vi "VIH Platform - Windows - SHELL Error Handler.vi"(8 "error in":errorcluster, 11 "SHELL Error Code":i32) -> (0 "error out":errorcluster)   [LabVIEW 2014]
doc: "::: VI Helpeks :::\nCopyright (c) 2000-2026 Konstantin Shifershteyn. All rights reserved."
panel:
  # "VI Helpeks\nCopyright (c) 2012-2026 Konstantin Shifershteyn"
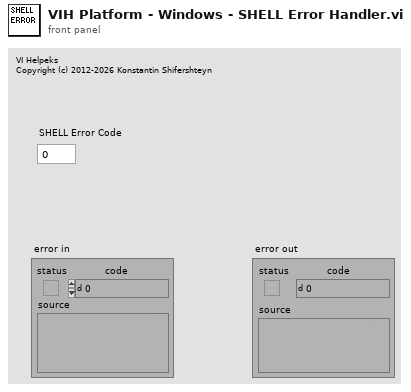
[diagram p1: front panel]
types:
  T1 = cluster{"Product Name":string, "Short Name":string, "Product Version":string, "Release Timestamp":string, "Developer":string, "Copyright":string}
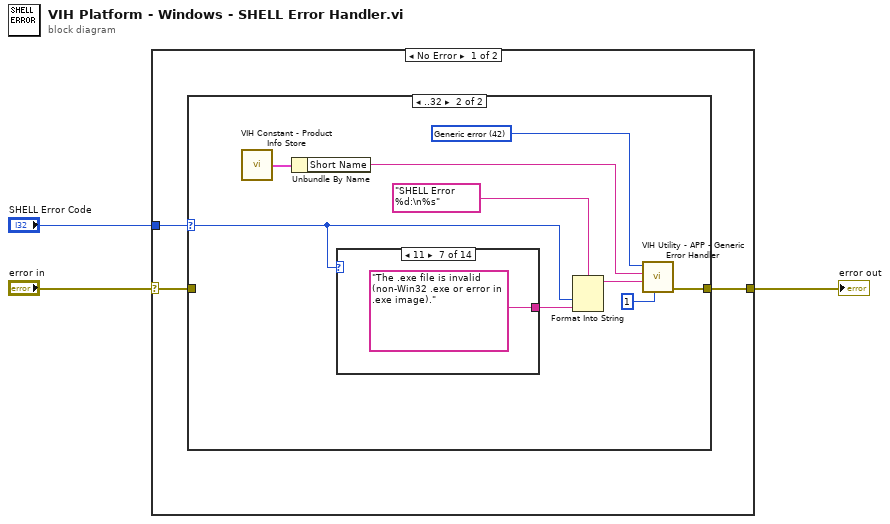
[diagram p0: block diagram]
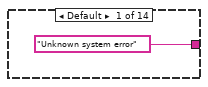
[diagram p3: hidden frame]
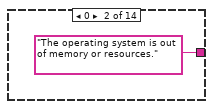
[diagram p4: hidden frame]
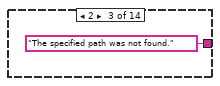
[diagram p5: hidden frame]
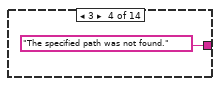
[diagram p6: hidden frame]
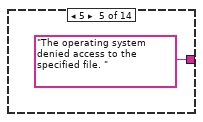
[diagram p7: hidden frame]
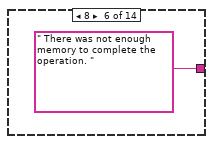
[diagram p8: hidden frame]
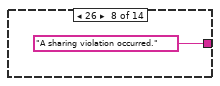
[diagram p9: hidden frame]
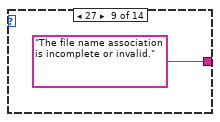
[diagram p10: hidden frame]
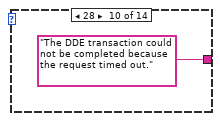
[diagram p11: hidden frame]
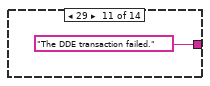
[diagram p12: hidden frame]
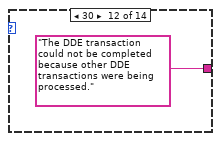
[diagram p13: hidden frame]
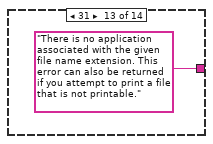
[diagram p14: hidden frame]
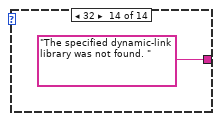
[diagram p15: hidden frame]
diagram:
  n1 = case shown="No Error" "error in" {
    selector: "error in" -> [w4 w31]
    tunnel: [w6 w31] -> w3
    tunnel: "SHELL Error Code" -> [w5 _]
    frame No Error {
      n2 = case shown="..32" w5 {
        selector: w5 -> [_ w11]
        tunnel: [w7 w15] -> w6
        tunnel: w4 -> [w7 _]
        frame Default {
        }
        frame ..32 {
          w16 = 42 items=["No error", "Argument error", "Memory is full", "Out of zone", "End of file", "File already open", "Generic file I/O error", "File not found", "File permission error", "Disk is full", "Duplicate path", "Too many files open", "System feature not enabled", "Resource file not found", "Cannot add resource", "Resource not found", "Image not found", "Image memory error", "Pen does not exist", "Config type invalid", "Config token not found", "Config parse error", "Config memory error", "Bad external code format", "Bad external code offset", "External code not present", "Null window", "Destroy window error", "Null menu", "Print aborted", "Bad print record", "Print driver error", "Windows error during printing", "Memory error during printing", "Print dialog error", "Generic print error", "Invalid device refnum", "Device not found", "Device parameter error", "Device unit error", "Cannot open device", "Device call aborted", "Generic error", "Cancelled by user", "Object ID too low", "Object ID too high", "Object not in heap", "Unknown heap", "Unknown object (invalid DefProc)", "Unknown object (DefProc not in table)", "Message out of range", "Invalid (null) method", "Unknown message", "Manager call not supported", "Bad address", "Network operation in progress", "Network operation timed out", "Connection is busy", "Network attribute not supported", "Network error", "Address in use", "System out of memory", "Connection aborted", "Connection refused", "Not connected", "Already connected", "Connection closed", "Initialization error (interapplication manager)", "Bad occurrence", "Wait on unbound occurrence handler", "Occurrence queue overflow", "Datalog type conflict", "Unused", "Unrecognized type (interapplication manager)", "Memory corrupt", "Failed to make temporary DLL", "Old CIN version", "Drag socket not found", "Failed to load drop-object", "Failed to register OLE object", "Failed to release OLE object", "Format specifier type mismatch", "Unknown format specifier", "Too few format specifiers", "Too many format specifiers", "Scan failed", "Newer CIN version", "Error converting to variant", "Runtime menu error", "Password tampered", "Variant attribute not found", "Incompatible variant data type", "Event data is not available", "Event Store is not present", "Occurrence is not found", "Event Queue is not created", "Event info is not available in the type library", "Refnum passed is NULL", "Error retrieving Class GUID", "Error retrieving CoClass GUID", "Error retrieving TypeLib GUID.", "Bad built application magic bytes.", "Specific driver is different from the specific driver associated with the Logical Name.", "There is no session opened to the class driver.", "Max Error", "MAX - Error with config objects", "MAX - Error loading configuration", "MAX - Group not supported", "Singlecast connections can not send to multicast addresses.", "Multicast connections can not send to singlecast addresses.", "Specified IP address not in multicast address range.", "Attempt to write to read-only multicast connection.", "Attempt to read from write-only multicast connection.", "The buffer used to receive a datagram was smaller than the datagram itself"]
          n3 = call "VIH Constant - Product Info Store.vi"() -> ("Product Info"=w9:T1)
          n4 = Unbundle By Name(w9) -> ("Short Name"=w8:string)
          n5 = case shown="11" w11 {
            tunnel: ["Unknown system error" "The operating system is out of memory or resources." "The specified path was not found." "The specified path was not found." "The operating system denied access to the specified file. " " There was not enough memory to complete the operation. " "The .exe file is invalid (non-Win32 .exe or error in .exe image)." "A sharing violation occurred." "The file name association is incomplete or invalid." "The DDE transaction could not be completed because the request timed out." "The DDE transaction failed." "The DDE transaction could not be completed because other DDE transactions were being processed." "There is no application associated with the given file name extension. This error can also be returned if you attempt to print a file that is not printable." "The specified dynamic-link library was not found. "] -> w13
            frame Default {
            }
            frame 0 {
            }
            frame 2 {
            }
            frame 3 {
            }
            frame 5 {
            }
            frame 8 {
            }
            frame 11 {
            }
            frame 26 {
            }
            frame 27 {
            }
            frame 28 {
            }
            frame 29 {
            }
            frame 30 {
            }
            frame 31 {
            }
            frame 32 {
            }
          }
          n6 = Format Into String(format string="SHELL Error %d:\n%s", w11, w13) -> (resulting string=w12:string)  [unwired: 2 in, 1 out]
          n7 = call "VIH Utility - APP - Generic Error Handler.vi"("nesting level"=1, "error reason"=w12, "error location"=w8, "error code"=w16) -> ("error out"=w15:errorcluster)  [unwired: 1 in, 6 out]
        }
      }
    }
    frame Error {
    }
  }
  "error out" <- w3
